vi "PicoScope5000aWrapSettings.vi"(1 "enabled array":i16[](array[numeric]), 8 "Device Info":T1, 10 "Handle In":i16, 11 "error in (no error)":errorcluster) -> (2 "Handle Out":i16, 3 "error out":errorcluster)   [LabVIEW 2010]
uses:
  ps5000aWrap.dll
  ps5000a.dll
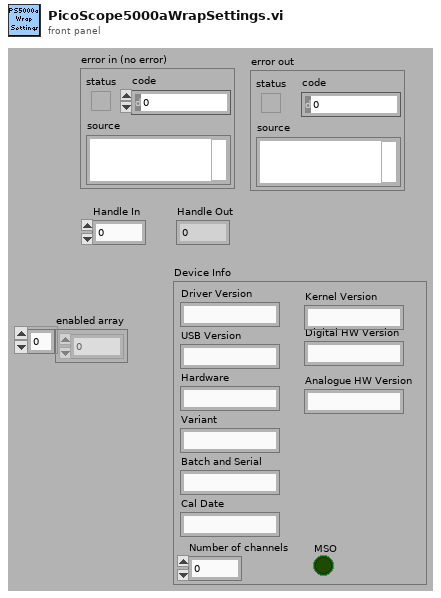
[diagram p1: front panel]
types:
  T1 = cluster{"Driver Version":string, "USB Version":string, "Hardware":string, "Variant":string, "Batch and Serial":string, "Cal Date":string, "Kernel Version":string, "Digital HW Version":string, "Analogue HW Version":string, "MSO":bool, "Number of channels":i16}
  T2 = cluster{"status":bool, "code":u32, "source":string}
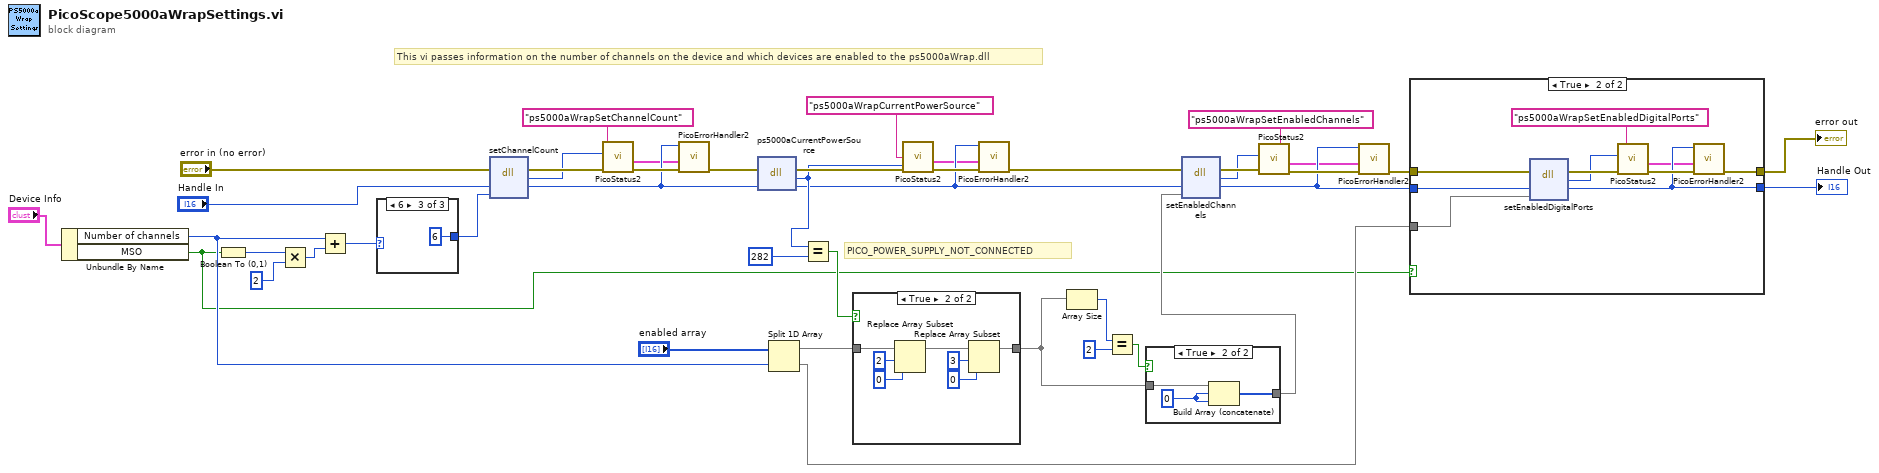
[diagram p0: block diagram]
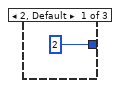
[diagram p5: hidden frame]
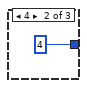
[diagram p6: hidden frame]
diagram:
  # "PICO_POWER_SUPPLY_NOT_CONNECTED"
  # "This vi passes information on the number of channels on the device and which devices are enabled to the ps5000aWrap.dll"
  n1 = Unbundle By Name("Device Info") -> ("Number of channels"=w10:i16, "MSO"=w4:bool)
  n2 = Boolean To (0,1)(Boolean=w4) -> (0, 1=w37:i16)
  n3 = Multiply(x=w37, y=i16 2) -> (x*y=w35:i16)
  n4 = Add(x=w10, y=w35) -> (x+y=w38:i16)
  n5 = case shown="6" w38 {
    tunnel: [i16 2 i16 4 i16 6] -> w41
    frame 2, Default {
    }
    frame 4 {
    }
    frame 6 {
    }
  }
  n6 = dll-call lib="ps5000aWrap.dll" fn="setChannelCount"(error in="error in (no error)", "handle"="Handle In", "channelCount"=w41) -> (error out=w20:errorcluster, "PICO_STATUS"=w17:u32, "handle"=w16:i16)  [unwired: 3 in, 1 out]
  n7 = call "PicoStatus2.vi"("PICO source"="ps5000aWrapSetChannelCount" ("source"), "Error in"=w20, "PICO STATUS"=w17) -> ("error out"=w22:errorcluster, "PICO_STATUS out"=w3:T2)  [unwired: 5 in]
  n8 = call "PicoErrorHandler2.vi"("error in (no error)"=w22, "PICO_STATUS in"=w3, "handle In"=w16) -> ("error out"=w18:errorcluster)  [unwired: 8 in]
  n9 = dll-call lib="ps5000a.dll" fn="ps5000aCurrentPowerSource"(error in=w18, "handle"=w16) -> (error out=w33:errorcluster, "PICO STATUS"=w24:u32, "handle"=w23:i16)  [unwired: 2 in, 1 out]
  n10 = Split 1D Array(array="enabled array", index=w10) -> (first subarray=w26:i16[], second subarray=w28:i16[])
  n11 = Equal?(x=w24, y=u32 282) -> (x = y?=w25:bool)
  n12 = case shown="True" w25 {
    tunnel: [w47 w53] -> w6
    tunnel: w26 -> [w47 w52]
    frame False {
    }
    frame True {
      n13 = Replace Array Subset(array=w52, new element=i16 0 ("new element/subarray"), index=2) -> (w54:i16[])
      n14 = Replace Array Subset(array=w54, new element=i16 0 ("new element/subarray"), index=3) -> (w53:i16[])
    }
  }
  n15 = call "PicoStatus2.vi"("PICO source"="ps5000aWrapCurrentPowerSource" ("source"), "Error in"=w33, "PICO STATUS"=w24) -> ("error out"=w32:errorcluster, "PICO_STATUS out"=w1:T2)  [unwired: 5 in]
  n16 = call "PicoErrorHandler2.vi"("error in (no error)"=w32, "PICO_STATUS in"=w1, "handle In"=w23) -> ("error out"=w31:errorcluster)  [unwired: 8 in]
  n17 = Array Size(array=w6) -> (size(s)=w7:i32)
  n18 = Equal?(x=w7, y=2) -> (x = y?=w8:bool)
  n19 = case shown="True" w8 {
    tunnel: w6 -> [w55 w58]
    tunnel: [w55 w56] -> w5
    frame False {
    }
    frame True {
      w57 = i16 0 ("y")
      n20 = Build Array (concatenate)(w58, w57, w57) -> (w56:i16[])
    }
  }
  n21 = dll-call lib="ps5000aWrap.dll" fn="setEnabledChannels"(error in=w31, "handle"=w23, "enabledChannels"=w5) -> (error out=w15:errorcluster, "PICO_STATUS"=w13:u32, "handle"=w11:i16)  [unwired: 3 in, 1 out]
  n22 = call "PicoStatus2.vi"("PICO source"="ps5000aWrapSetEnabledChannels" ("source"), "Error in"=w15, "PICO STATUS"=w13) -> ("error out"=w21:errorcluster, "PICO_STATUS out"=w2:T2)  [unwired: 5 in]
  n23 = call "PicoErrorHandler2.vi"("error in (no error)"=w21, "PICO_STATUS in"=w2, "handle In"=w11) -> ("error out"=w12:errorcluster)  [unwired: 8 in]
  n24 = case shown="True" w4 {
    tunnel: w12 -> [w60 w70]
    tunnel: w11 -> [w59 w69]
    tunnel: [w60 w63] -> w30
    tunnel: [w59 w62] -> w29
    tunnel: w28 -> [_ w68]
    frame False {
    }
    frame True {
      n25 = dll-call lib="ps5000aWrap.dll" fn="setEnabledDigitalPorts"(error in=w70, "handle"=w69, "enabledChannels"=w68) -> (error out=w66:errorcluster, "PICO_STATUS"=w64:u32, "handle"=w62:i16)  [unwired: 3 in, 1 out]
      n26 = call "PicoStatus2.vi"("PICO source"="ps5000aWrapSetEnabledDigitalPorts" ("source"), "Error in"=w66, "PICO STATUS"=w64) -> ("error out"=w67:errorcluster, "PICO_STATUS out"=w61:T2)  [unwired: 5 in]
      n27 = call "PicoErrorHandler2.vi"("error in (no error)"=w67, "PICO_STATUS in"=w61, "handle In"=w62) -> ("error out"=w63:errorcluster)  [unwired: 8 in]
    }
  }
  "Handle Out" <- w29
  "error out" <- w30
